vi "Create.vi"(7 "Request Options":T1={"request headers"=[], "request parameters"=[], "request body"="", "region handling"=enum."use region everywhere", "URL formatting"=enum."region."}, 8 "error in (no error)":errorcluster, 9 "Region":T5, 10 "AWS Credentials":T6, 11 "ARN in":refnum<class "ARN.lvclass">) -> (0 "error out":errorcluster, 3 "ARN out":refnum<class "ARN.lvclass">)   [LabVIEW 2015, in "NI_AWS_Core.lvlib" / "ARN.lvclass"]
uses:
  ARN.lvclass
  XML Parsing/NI_XML Parsing.lvlib
  HTTP Request/HTTP Request.lvclass
  HTTP Request/AWS Credentials.ctl
  HTTP Request/Region.ctl
  HTTP Request/Name Value Pair.ctl
  HTTP Request/Request Options.ctl
  HTTP Request/Region handling.ctl
  HTTP Request/URL formatting.ctl
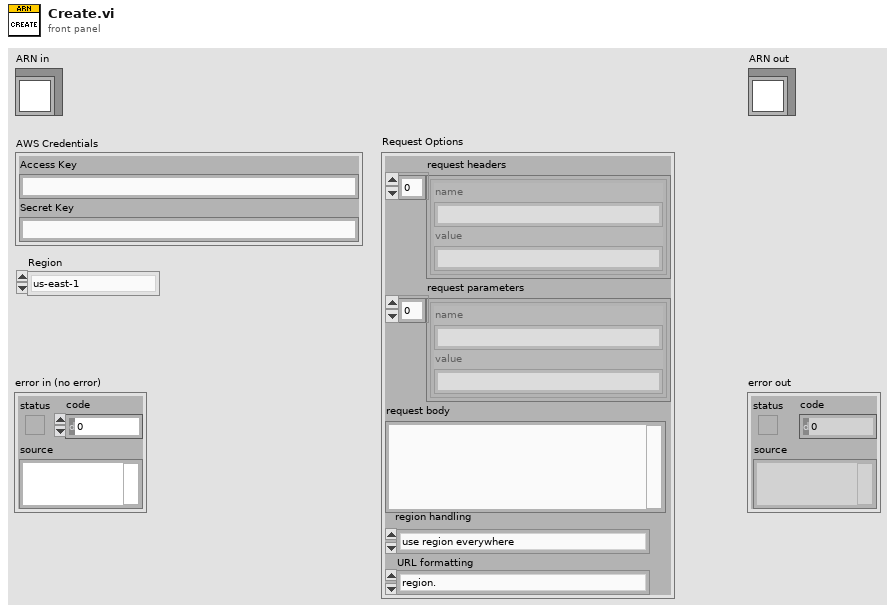
[diagram p1: front panel]
types:
  T1 = typedef "NI_AWS_Core.lvlib/HTTP Request.lvclass/Request Options.ctl" = cluster{"request headers":T2[], "request parameters":T2[], "request body":string, "region handling":T3, "URL formatting":T4}
  T2 = typedef "NI_AWS_Core.lvlib/HTTP Request.lvclass/Name Value Pair.ctl" = cluster{"name":string, "value":string}
  T3 = typedef "NI_AWS_Core.lvlib/HTTP Request.lvclass/Region handling.ctl" = enum16{"use region everywhere", "use region (authentication only)", "use region (URL only)", "ignore region everwhere"}
  T4 = typedef "NI_AWS_Core.lvlib/HTTP Request.lvclass/URL formatting.ctl" = enum16{"region-", "region."}
  T5 = typedef "NI_AWS_Core.lvlib/HTTP Request.lvclass/Region.ctl" = enum16{"us-east-1", "us-east-2", "us-west-1", "us-west-2", "ap-northeast-1", "ap-northeast-2", "ap-southeast-1", "ap-southeast-2", "ca-central-1", "eu-central-1", "eu-west-1", "eu-west-2", "sa-east-1"}
  T6 = typedef "NI_AWS_Core.lvlib/HTTP Request.lvclass/AWS Credentials.ctl" = cluster{"Access Key":string, "Secret Key":string}
  T7 = typedef "NI_AWS_Core.lvlib/HTTP Request.lvclass/Response.ctl" = cluster{"Headers":string, "Body":string}
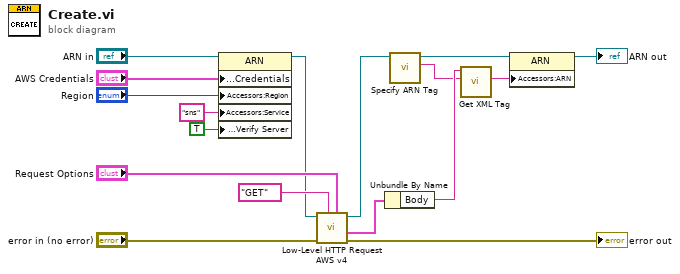
[diagram p0: block diagram]
diagram:
  n1 = property class="ARN"(reference="ARN in", "Accessors:Credentials"="AWS Credentials", "Accessors:Region"="Region", "Accessors:Service"="sns" ("Service"), "Accessors:Verify Server"=TRUE ("Verify Server")) -> (reference out=w2:refnum<class "ARN.lvclass">)  [unwired: 1 in, 1 out]
  n2 = call "Low-Level HTTP Request AWS v4.vi"("Request Options"="Request Options", "HTTP-Verb"="GET", "error in (no error)"="error in (no error)", "AWS Core in"=w2) -> ("error out"=→"error out":errorcluster, "Response"=w3:T7, "AWS Core out"=w1:refnum<class "ARN.lvclass">)  [unwired: 4 in, 1 out]
  n3 = Unbundle By Name(w3) -> ("Body"=w17:string)
  n4 = call-dynamic "Specify ARN Tag.vi"("ARN in"=w1) -> ("ARN Tag"=w6:string, "ARN out"=w7:refnum<class "ARN.lvclass">)  [unwired: 9 in]
  n5 = call "Get XML Tag.vi"("Tag name"=w6, "XML String in"=w17) -> ("Tag value"=w12:string)  [unwired: 5 in, 4 out]
  n6 = property class="ARN"(reference=w7, "Accessors:ARN"=w12) -> (reference out=→"ARN out":refnum<class "ARN.lvclass">)  [unwired: 1 in, 1 out]
